vi "Send Exit Message to UI MHL.vi"(8 "error in (no error)":errorcluster, 11 "Message Queues":T1) -> (0 "error out":errorcluster)   [LabVIEW 2020, in "MHL Templete.lvlib"]
doc: "すべてのメッセージキューにExitメッセージを送る。"
uses:
  MHL Templete.lvlib
  e7f3e565-3e0e-48e1-9954-56ed745e6014.vi
  support/Message Queue/Message Cluster.ctl
  support/Message Queue/Message Queue.lvlib
  support/Message Queue/All Message Queues.ctl
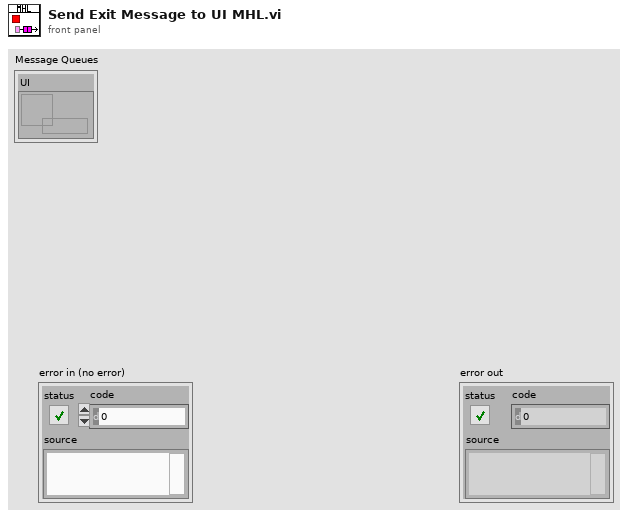
[diagram p1: front panel]
types:
  T1 = typedef "Message Queue.lvlib/All Message Queues.ctl" = cluster{"UI":refnum<queue>}
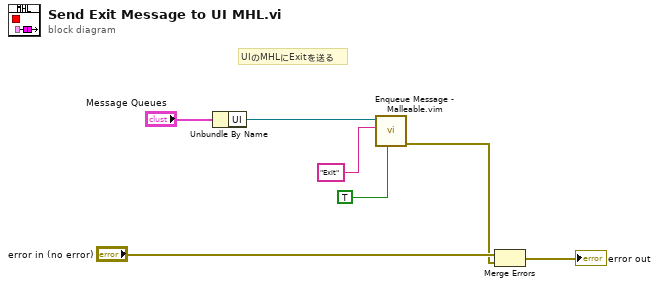
[diagram p0: block diagram]
diagram:
  # "UIのMHLにExitを送る"
  n1 = Unbundle By Name("Message Queues") -> ("UI"=w6:refnum<queue>)
  n2 = call "Enqueue Message - Malleable.vim"("Priority Message? (F)"=TRUE, "Message"="Exit", "Message Queue"=w6) -> ("error out"=w3:errorcluster)  [unwired: 7 in, 1 out]
  n3 = Merge Errors("error in (no error)", w3) -> (→"error out":errorcluster)
